vi "Transport_Heartbeat.vi"(8 "error in (no error)":errorcluster={"status"=FALSE, "code"=0, "source"="\"\""}, 10 "monotonic clock":string, 11 "Link status":string) -> (0 "error out":errorcluster={"status"=FALSE, "code"=0, "source"="\"\""}, 2 "status ok":bool, 3 "Heartbeat events":string)   [LabVIEW 2026]
doc: "INTENT: Maintain connectivity health. LOGIC: Transmit and monitor heartbeat sequence independently of operator prompts."
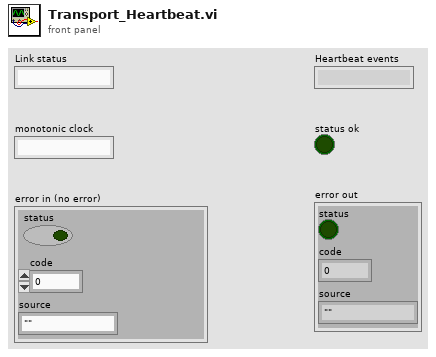
[diagram p1: front panel]
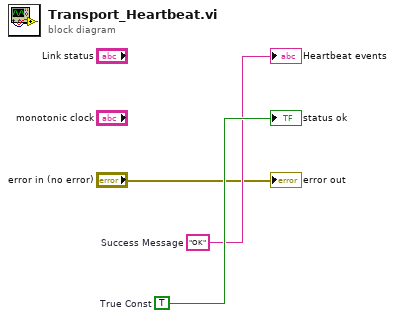
[diagram p0: block diagram]
diagram:
  w3 = TRUE  # True Const
  w2 = "OK"  # Success Message
  "Heartbeat events" <- w2
  "status ok" <- w3
  "error out" <- "error in (no error)"
